vi "Add Error to Display.vi"(8 "error in (no error)":errorcluster, 10 "error to display":T1 {"Time Stamp" format="%<%x %.3X>T"}, 11 "Error Manager in":refnum<class "Error Manager.lvclass">) -> (0 "error out":errorcluster, 3 "Error Manager out":refnum<class "Error Manager.lvclass">)   [LabVIEW 2020, in "TALOS.lvlib" / "Error Manager.lvlib" / "Error Manager.lvclass"]
uses:
  Error Manager.lvclass
  C:/Users/marco/Documents/GitHub_Lab/TALOS/talos/Father of all uServices/Father of all uServices/Father of all uServices.lvclass
  Error Info.ctl
  Common GUI v3/Common GUI v3/Error Listbox Msg.ctl
  Common GUI v3/Common GUI v3/Error Listbox Msg Action.ctl
  Error Manager.lvclass/Error Manager.ctl
  Father of all uServices/Father of all uServices/Father of all uServices.lvclass/Father of all uServices.ctl
  Ancestor/Ancestor/Ancestor.lvclass/Ancestor.ctl
  Guardian/Guardian/Requests.ctl
  Guardian/Guardian Messages/Requests from uServices Msg/Requests from uServices Msg.lvclass/Requests from uServices Msg.ctl
  Support VIs/Substitute Error.vi
  Guardian/Guardian Messages/Requests from uServices Msg/Send Requests from uServices.vi
  Support VIs/Generate Error.vi
  FGV/Error Memory/Get Error Description.vi
  Support VIs/Get PC name.vi
  Ancestor/Ancestor/Read ID.vi
  Support VIs/Get Class Name.vi
  <vilib>/Utility/error.llb/Clear Errors.vi
  FGV/Error Memory/Error Memory Core.vi
  <vilib>/AdvancedString/Delimited String to 1D String Array.vi
  Support VIs/Circus Root Path.vi
  FGV/Error Memory/Error Crt Lvl checker.vi
  FGV/Error Memory/Error Memory Core.vi/40c8088d-b597-4017-91af-faa98e00292e.vi
  FGV/Error Memory/Error Memory Core.vi/d4a3ab98-063c-4e44-b43d-fbdcfe6c2be2.vi
  Father of all uServices/Father of all uServices/Father of all uServices.lvclass
  C:/Users/marco/Documents/GitHub_Lab/TALOS/builds/Actor Framework PPL/Actor Framework.lvlibp/1abvi3w/vi.lib/ActorFramework/Actor/Actor.lvclass
  Support VIs/Global Memory.vi
  Support VIs/Global Constants.vi
  <vilib>/Utility/LVClass/Get LV Class Name.vi
  Support VIs/Is in Packed Library.vi
  Support VIs/TALOS Root path.vi
  Support VIs/Read CSV worksheet.vi
  <vilib>/Utility/error.llb/General Error Handler.vi
  Support VIs/Error Log.vi
  builds/Actor Framework PPL/Actor Framework.lvlibp/1abvi3w/vi.lib/ActorFramework/Actor/Read Caller Enqueuer.vi
  builds/Actor Framework PPL/Actor Framework.lvlibp/1abvi3w/vi.lib/ActorFramework/Message Enqueuer/Enqueue.vi
  Ancestor/Ancestor/Ancestor.lvclass
  <vilib>/Comparison/Equal/Equal Functor/Equal Functor.lvclass
  Guardian/Guardian Messages/Requests from uServices Msg/Requests from uServices Msg.lvclass
  Guardian/Guardian/Guardian.lvclass
  Common GUI v3/Common GUI v3/Common GUI v3.lvclass
  TALOS.lvlib
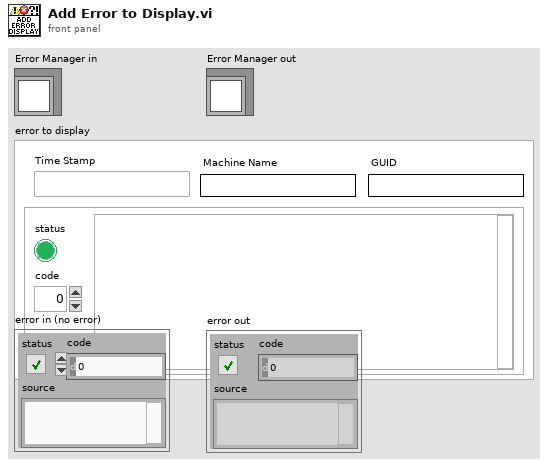
[diagram p1: front panel]
types:
  T1 = typedef "TALOS.lvlib/Error Manager.lvlib/Error Manager.lvclass/Error Info.ctl" = cluster{"error out":errorcluster, "Time Stamp":timestamp, "Machine Name":string, "GUID":string}
  T2 = typedef "TALOS.lvlib/Common GUI v3.lvlib/Common GUI v3.lvclass/Error Listbox Msg.ctl" = cluster{"Action":T3, "Error Info":T1}
  T3 = typedef "TALOS.lvlib/Common GUI v3.lvlib/Common GUI v3.lvclass/Error Listbox Msg Action.ctl" = enum16{"Add", "Remove", "Clear"}
  T4 = typedef "TALOS.lvlib/Guardian.lvlib/Guardian.lvclass/Requests.ctl" = enum16{"Ready to Launch", "Start RUN", "Stop RUN", "Update DAQ Params", "Update Error Listbox", "Update Run Status", "Update Kasli Log", "Run Stopped with Errors", "Switch uS View"}
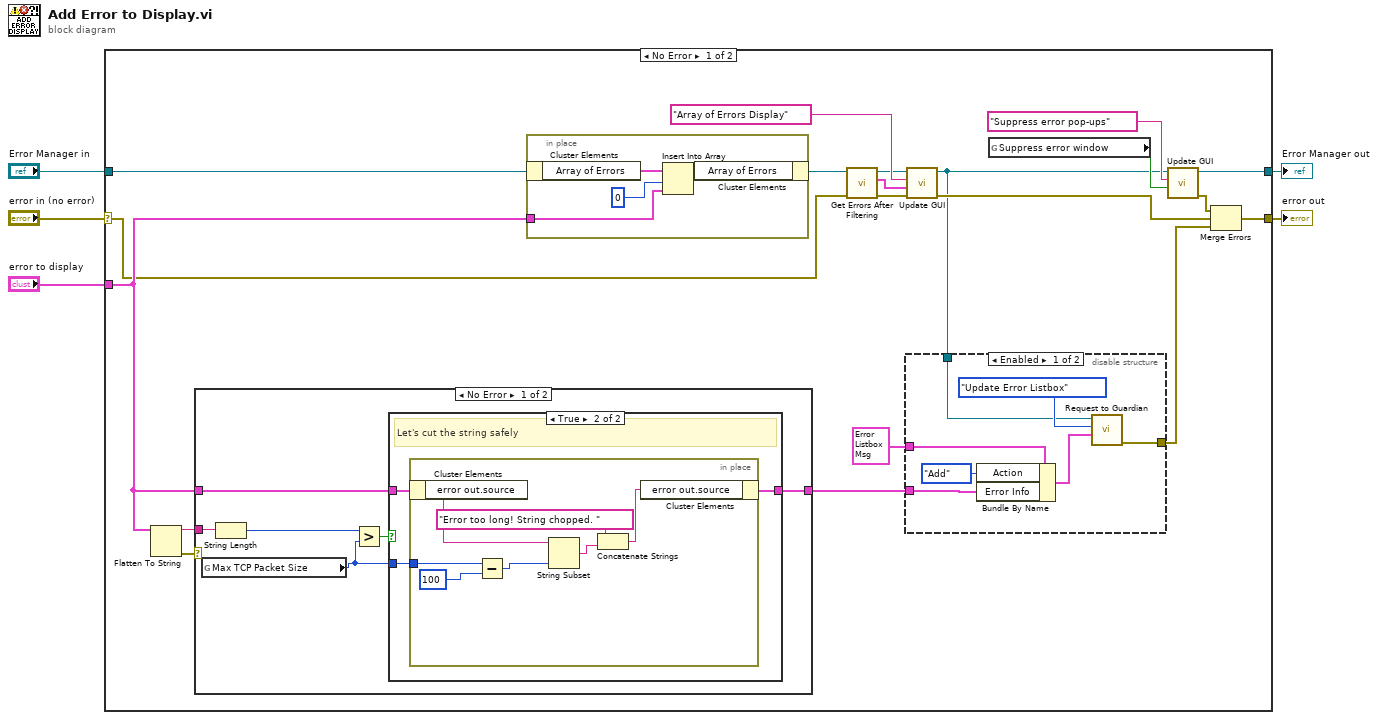
[diagram p0: block diagram]
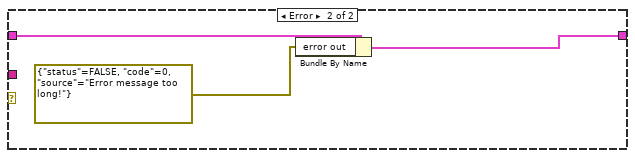
[diagram p3: hidden frame]
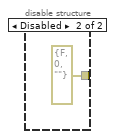
[diagram p4: hidden frame]
diagram:
  n1 = case shown="No Error" "error in (no error)" {
    selector: "error in (no error)" -> [w7 w59]
    tunnel: [w18 w58] -> w5
    tunnel: "error to display" -> [w12 _]
    tunnel: "Error Manager in" -> [w14 w58]
    tunnel: [w24 w59] -> w1
    frame No Error {
      n2 = Flatten To String(anything=w12) -> (data string=w22:string, error out=w21:errorcluster)  [unwired: 3 in, 1 out]
      n3 = case shown="No Error" w21 {
        tunnel: w22 -> [w35 _]
        tunnel: w12 -> [w33 w49]
        tunnel: [w31 w48] -> w20
        frame No Error {
          n4 = global read "Global Constants.vi" "Max TCP Packet Size"() -> (w30:u16)
          n5 = String Length(string=w35) -> (length=w34:i32)
          n6 = Greater?(x=w34, y=w30) -> (0:w32:bool)
          n7 = case shown="True" w32 {
            tunnel: w33 -> [w36 w39]
            tunnel: [w36 w38] -> w31
            tunnel: w30 -> [_ w37]
            frame False {
              # "Length OK, send it."
            }
            frame True {
              # "Let's cut the string safely"
              n8 = in-place {
                in-place-border: w37 -> [w45]
                n9 = in-place-cluster #1(w39) -> ("error out.source"=w46:string)
                n10 = Subtract(x=w45, y=u16 100) -> (x-y=w43:u16)
                n11 = String Subset(string=w46, length (rest)=w43) -> (substring=w42:string)  [unwired: 1 in]
                n12 = Concatenate Strings("Error too long! String chopped. " ("source"), w42) -> (w40:string)
                n13 = in-place-cluster #1("error out.source"=w40) -> (w38:T1)
              }
            }
          }
        }
        frame Error {
          n14 = Bundle By Name(cluster=w49, "error out"=errorcluster {"status"=FALSE, "code"=0, "source"="Error message too long!"}) -> (w48:T1)
        }
      }
      n15 = in-place {
        in-place-border: w12 -> [w27]
        n16 = in-place-cluster #2(w14) -> ("Array of Errors"=w29:T1[])
        n17 = Insert Into Array(array=w29, index=0, new element=w27) -> (w28:T1[])
        n18 = in-place-cluster #2("Array of Errors"=w28) -> (w13:refnum<class "Error Manager.lvclass">)
      }
      n19 = call-dynamic "Get Errors After Filtering.vi"("error in (no error)"=w7, "Error Manager in"=w13) -> ("error out"=w8:errorcluster, "Array of Errors"=w9:T1[], "Error Manager out"=w10:refnum<class "Error Manager.lvclass">)  [unwired: 7 in]
      n20 = call "Update GUI.vi"("error in (no error)"=w8, "Data"=w9, "GUI Item Name"="Array of Errors Display" ("FP Item Name"), "uService Template in"=w10) -> ("error out"=w19:errorcluster, "uService Template out"=w6:refnum<class "Error Manager.lvclass">)  [unwired: 6 in]
      n21 = disable-structure shown="Enabled" {
        disable-tunnel: T2 {"Action"=enum."Add", "Error Info"={"error out"={"status"=FALSE, "code"=0, "source"=""}, "Time Stamp"=timestamp(0 s since 1904-01-01), "Machine Name"="", "GUID"=""}} ("Error Listbox Msg") -> [w55 _]
        disable-tunnel: w20 -> [w53 _]
        disable-tunnel: [w51 errorcluster {"status"=FALSE, "code"=0, "source"=""} ("error out")] -> w23
        disable-tunnel: w6 -> [w50 _]
        frame Enabled {
          n22 = Bundle By Name(cluster=w55, "Action"=Error_Listbox_Msg_Action."Add", "Error Info"=w53) -> (w52:T2)
          n23 = call "Request to Guardian.vi"("Data"=w52, "Requests"=Requests."Update Error Listbox", "Father of all uServices in"=w50) -> ("error out"=w51:errorcluster)  [unwired: 7 in, 1 out]
        }
        frame Disabled {
        }
      }
      n24 = global read "Global Memory.vi" "Suppress error window"() -> (w15:bool)
      n25 = call "Update GUI.vi"("Data"=w15, "GUI Item Name"="Suppress error pop-ups", "uService Template in"=w6) -> ("error out"=w17:errorcluster, "uService Template out"=w18:refnum<class "Error Manager.lvclass">)  [unwired: 7 in]
      n26 = Merge Errors(w17, w19, w23) -> (w24:errorcluster)
    }
    frame Error {
    }
  }
  "Error Manager out" <- w5
  "error out" <- w1
